vi "Create Services.vi"(8 "error in (no error)":errorcluster, 10 "NI GUID":string, 11 "gRPC server in":refnum<class "Servicer.lvclass">) -> (0 "error out":errorcluster, 2 "gRPC services out":refnum<class "ServiceBase.lvclass">[](array[class]), 3 "gRPC server out":refnum<class "Servicer.lvclass">)   [LabVIEW 2025, in "OOB gRPC Server.lvlib"]
uses:
  OOB gRPC Server.lvlib
  <vilib>/gRPC/LabVIEW gRPC Servicer/Servicer/Servicer.lvclass
  <vilib>/gRPC/LabVIEW gRPC Servicer/ServiceBase/ServiceBase.lvclass
  <vilib>/gRPC/LabVIEW gRPC Servicer/Servicer/Servicer.lvclass/Servicer.ctl
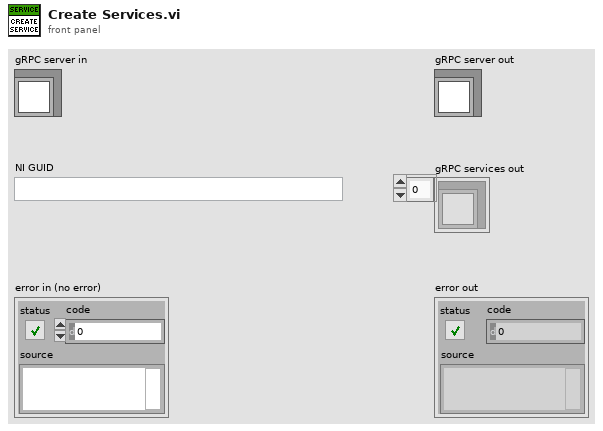
[diagram p1: front panel]
types:
  T1 = typedef "grpc-lvsupport-release.lvlib/grpcId.ctl" = u64
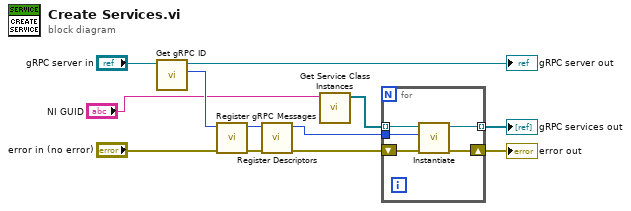
[diagram p0: block diagram]
diagram:
  n1 = call <vilib>:"Get gRPC ID.vi"("gRPC server in"="gRPC server in") -> ("gRPC ID"=w12:T1, "gRPC server out"=→"gRPC server out":refnum<class "Servicer.lvclass">)  [unwired: 9 in]
  n2 = call "Register gRPC Messages.vi"("error in (no error)"="error in (no error)", "gRPC ID"=w12) -> ("error out"=w11:errorcluster, "gRPC ID Out"=w10:T1)  [unwired: 8 in]
  n3 = call "Register Descriptors.vi"("error in (no error)"=w11, "gRPC ID"=w10) -> ("error out"=w8:errorcluster, "gRPC ID Out"=w7:T1)  [unwired: 8 in]
  n4 = call "Get Service Class Instances.vi"("NI GUID"="NI GUID") -> ("service instances"=w6:refnum<class "ServiceBase.lvclass">[])  [unwired: 10 in]
  n5 = for {
    tunnel: w7 -> [w15]
    shift-right: [w14] -> w2
    shift-left: w8 -> [w16]
    tunnel: w6 -> [w17] mode=indexing
    tunnel: [w13] -> w3 mode=indexing
    n6 = call-dynamic "Instantiate.vi"("error in"=w16, "gRPCid"=w15, "gRPC service in"=w17) -> ("error out"=w14:errorcluster, "gRPC service out"=w13:refnum<class "ServiceBase.lvclass">)  [unwired: 7 in]
  }
  "error out" <- w2
  "gRPC services out" <- w3
